vi "Launch Detached.vi"(0 "path":path) -> (15 "error out":errorcluster)   [LabVIEW 2020]
doc: "Test helper: opens the front panel of the VI at path and runs it without waiting."
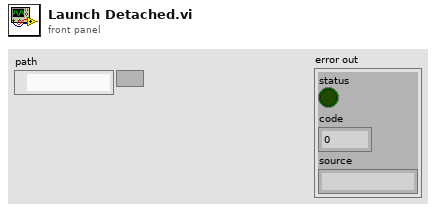
[diagram p1: front panel]
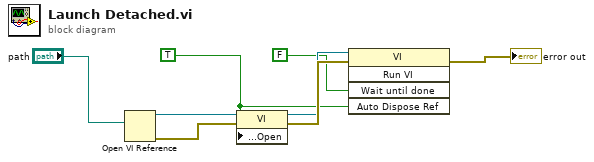
[diagram p0: block diagram]
diagram:
  w4 = TRUE
  n1 = Open VI Reference(vi path="path") -> (vi reference=w2:refnum<vi>, error out=w3:errorcluster)  [unwired: 5 in]
  n2 = property class="VI"(reference=w2, error in=w3, "Front Panel Window:Open"=w4) -> (reference out=w6:refnum<vi>, error out=w7:errorcluster)
  n3 = invoke class="VI" method="Run VI"(reference=w6, error in=w7, "Wait until done"=FALSE, "Auto Dispose Ref"=w4) -> (error out=→"error out":errorcluster)  [unwired: 1 in, 4 out]
